vi "[ex ce] XY Chart of two variables.vi"() -> ()   [LabVIEW 2021]
doc: "This simplest example evaluates two formulas and displays result in a XY chart.\n\n::: CalcExpress Toolkit :::\nCopyright (c) 2000-2026 Konstantin Shifershteyn. All rights reserved."
panel:
  in  "chart length (points)":i32=150
  in  "update period, ms":u32=10
  in  "stop":bool
  out "chart":cluster{dbl, dbl}[](graph)
  in  "Expression":string="x = sin(i) * sin(i/5);\ny = sin(i) * cos(i/5);\ni+= 0.1;"
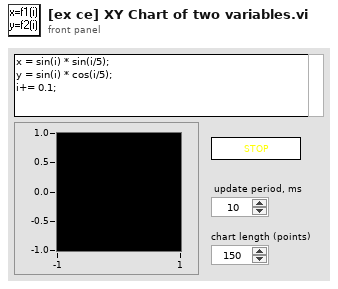
[diagram p1: front panel]
types:
  T1 = typedef "VarMan Variable Context Handle.ctl" = i32
  T2 = enum16{"create", "destroy", "set value", "get value"}
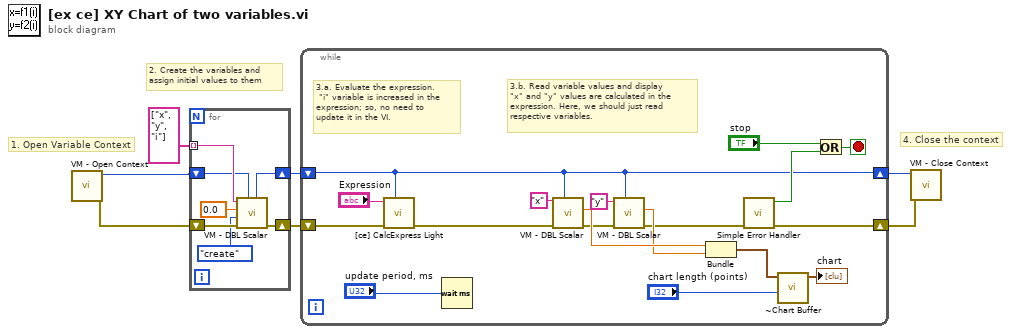
[diagram p0: block diagram]
diagram:
  # "4. Close the context"
  # "2. Create the variables and\nassign initial values to them"
  # "1. Open Variable Context"
  n1 = call "VM - Open Context.vi"() -> ("error out"=w7:errorcluster, "VC Handle out"=w5:T1)  [unwired: 9 in, 1 out]
  n2 = for {
    shift-right: [w13] -> w1
    shift-left: w7 -> [w14]
    tunnel: string[] ["x", "y", "i"] -> [w12] mode=indexing
    shift-right: [w9] -> w4
    shift-left: w5 -> [w10]
    n3 = call "VM - DBL Scalar.vi"("VC Handle"=w10, "error in"=w14, "cmd"=T2."create", "value in"=0.0 ("val (0)"), "name_spec"=w12) -> ("error out"=w13:errorcluster, "dup VC Handle"=w9:T1)  [unwired: 1 in, 4 out]
  }
  n4 = while {
    shift-right: [w15] -> w3
    shift-left: w4 -> [w15]
    shift-right: [w17] -> w2
    shift-left: w1 -> [w19]
    stop <- w31 stop-if-true
    # "3.b. Read variable values and display\n\"x\" and \"y\" values are calculated in the\nexpression. Here, we should just read\nrespective variables."
    # "3.a. Evaluate the expression.\n \"i\" variable is increased in the\nexpression; so, no need to\nupdate it in the VI."
    n5 = call "[ce] CalcExpress Light.vi"("VC Handle"=w15, "error in"=w19, "expression"="Expression") -> ("error out"=w20:errorcluster)  [unwired: 6 in, 2 out]
    n6 = Wait (ms)(milliseconds to wait="update period, ms") -> ()  [unwired: 1 out]
    n7 = call "VM - DBL Scalar.vi"("VC Handle"=w15, "error in"=w20, "name_spec"="x" ("var name")) -> ("error out"=w21:errorcluster, "value out"=w26:dbl)  [unwired: 3 in, 4 out]
    n8 = call "VM - DBL Scalar.vi"("VC Handle"=w15, "error in"=w21, "name_spec"="y" ("var name")) -> ("error out"=w18:errorcluster, "value out"=w25:dbl)  [unwired: 3 in, 4 out]
    n9 = Bundle("value out"=w26, "value out"=w25) -> (w27:cluster{"value out":dbl, "value out":dbl})  [unwired: 1 in]
    n10 = call <vilib>:"Simple Error Handler.vi"("error in (no error)"=w18) -> ("error?"=w16:bool, "error out"=w17:errorcluster)  [unwired: 4 in, 3 out]
    n11 = call "~Chart Buffer.vi"("buff size"="chart length (points)", "point"=w27) -> ("buff out"=→"chart":cluster{"x":dbl, "y":dbl}[])  [unwired: 9 in]
    n12 = Or(x="stop", y=w16) -> (x .or. y?=w31:bool)
  }
  n13 = call "VM - Close Context.vi"("error in"=w2, "VC Handle"=w3) -> ()  [unwired: 8 in, 2 out]
